vi "G-Parse-Uart_config.vi"(8 "error in (no error)":errorcluster caption="错误输入（无错误）", 10 "Data":string[][](array[string]), 11 "G-Uart-Class 输入":refnum<class "G-Uart-Class.lvclass">) -> (0 "error out":errorcluster caption="错误输出", 2 "配置数组":string[][](array[string]), 3 "G-Uart-Class 输出":refnum<class "G-Uart-Class.lvclass">)   [LabVIEW 2025, in "G-Uart-Class.lvclass"]
uses:
  G-Uart-Class.lvclass
  Register-Uart.ctl
panel:
  in  "Uart":T1
  # "启用终止符？"
  # "com口"
  # "波特率"
  # "数据位"
  # "停止位"
  # "奇偶校验"
  # "流控制"
  # "超时时间"
  # "终止符"
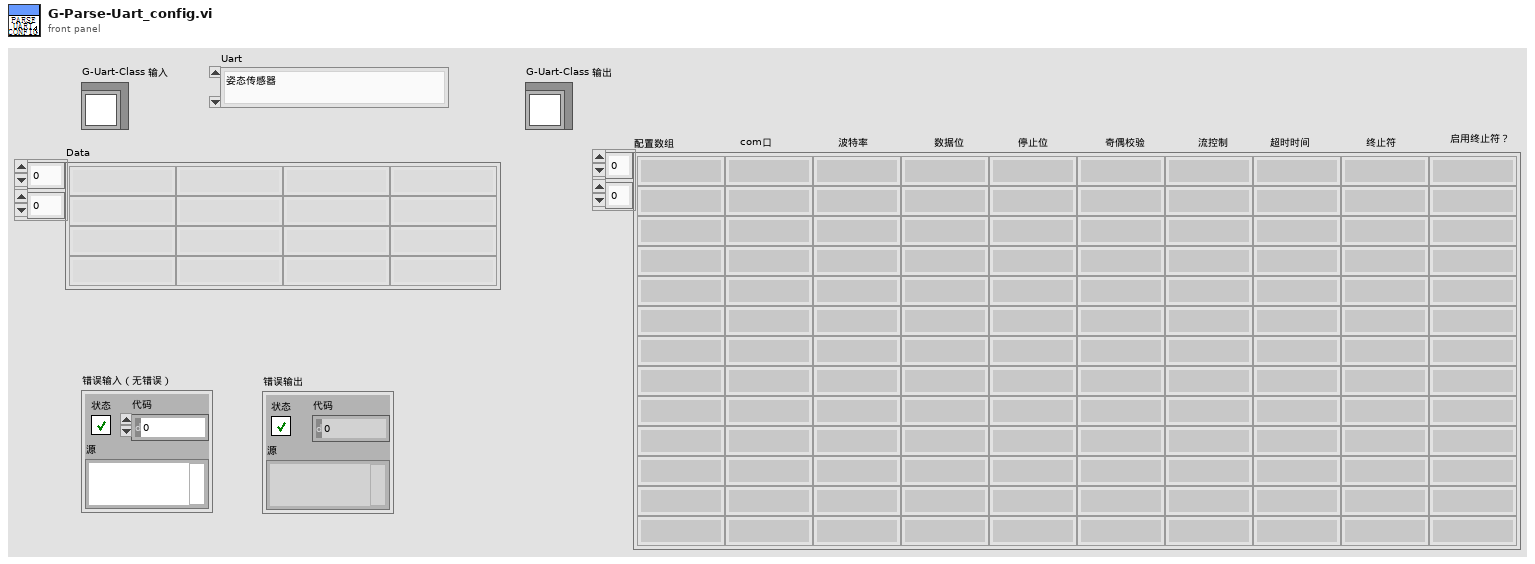
[diagram p1: front panel]
types:
  T1 = typedef "G-Uart-Class.lvclass/Register-Uart.ctl" = enum16{"姿态传感器", "图像跟踪", "观瞄仪器", "电源"}
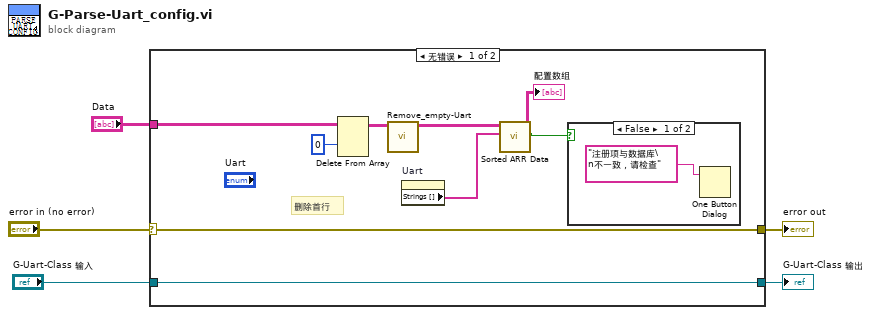
[diagram p0: block diagram]
diagram:
  n1 = case shown="无错误" "error in (no error)" {
    selector: "error in (no error)" -> [w13 w17]
    tunnel: [w13 w17] -> w4
    tunnel: [w14 w16] -> w2
    tunnel: "G-Uart-Class 输入" -> [w14 w16]
    tunnel: "Data" -> [w11 _]
    frame No Error {
      # "删除首行"
      n2 = Delete From Array(array=w11, index (row)=0 ("索引")) -> (array with subset deleted=w10:string[][])  [unwired: 2 in, 1 out]
      n3 = call "Remove_empty-Uart.vi"("ARR_in"=w10) -> ("ARR_out"=w9:string[][])  [unwired: 10 in]
      n4 = property on="Uart" class="Enum (严格)"() -> ("Strings []"=w6:string[])  [unwired: 2 in, 2 out]
      n5 = call "Sorted ARR Data.vi"("Uart-num"=w6, "Data"=w9) -> ("Consistent"=w8:bool, "Data-Sorted"=→"配置数组":string[][])  [unwired: 8 in]
      n6 = case shown="False" w8 {
        frame False {
          n7 = One Button Dialog(message="注册项与数据库\n不一致，请检查" ("消息")) -> ()  [unwired: 1 in, 1 out]
        }
        frame True {
        }
      }
    }
    frame Error {
    }
  }
  "error out" <- w4
  "G-Uart-Class 输出" <- w2
